vi "midiout_main.vi"() -> ()   [LabVIEW 2020]
uses:
  shared/midi note number.ctl
  midi/midi.lvclass
  0b612464-4594-4010-8acf-3e2bca421995.vi
  midi/midichannel.set.vi
  midi-ui/midi-ui.lvclass
panel:
  out "Currently Playing":T1
  out "2D Picture":picture
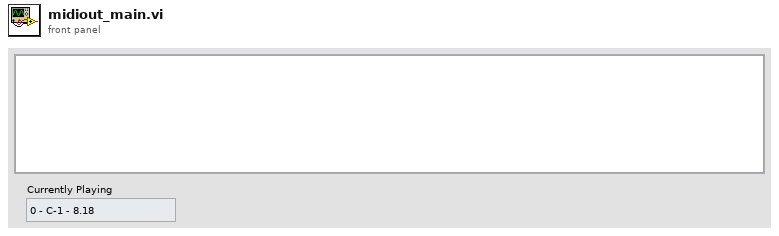
[diagram p1: front panel]
types:
  T1 = typedef "midi note number.ctl" = enum8{"0 - C-1 - 8.18", "1 - C#-1 - 8.66", "2 - D-1 - 9.18", "3 - D#-1 - 9.72", "4 - E-1 - 10.30", "5 - F-1 - 10.91", "6 - F#-1 - 11.56", "7 - G-1 - 12.25", "8 - G#-1 - 12.98", "9 - A-1 - 13.75", "10 - A#-1 - 14.57", "11 - B-1 - 15.43", "12 - C0 - 16.35", "13 - C#0 - 17.32", "14 - D0 - 18.35", "15 - D#0 - 19.45", "16 - E0 - 20.60", "17 - F0 - 21.83", "18 - F#0 - 23.12", "19 - G0 - 24.50", "20 - G#0 - 25.96", "21 - A0 - 27.50", "22 - A#0 - 29.14", "23 - B0 - 30.87", "24 - C1 - 32.70", "25 - C#1 - 34.65", "26 - D1 - 36.71", "27 - D#1 - 38.89", "28 - E1 - 41.20", "29 - F1 - 43.65", "30 - F#1 - 46.25", "31 - G1 - 49.00", "32 - G#1 - 51.91", "33 - A1 - 55.00", "34 - A#1 - 58.27", "35 - B1 - 61.74", "36 - C2 - 65.41", "37 - C#2 - 69.30", "38 - D2 - 73.42", "39 - D#2 - 77.78", "40 - E2 - 82.41", "41 - F2 - 87.31", "42 - F#2 - 92.50", "43 - G2 - 98.00", "44 - G#2 - 103.83", "45 - A2 - 110.00", "46 - A#2 - 116.54", "47 - B2 - 123.47", "48 - C3 - 130.81", "49 - C#3 - 138.59", "50 - D3 - 146.83", "51 - D#3 - 155.56", "52 - E3 - 164.81", "53 - F3 - 174.61", "54 - F#3 - 185.00", "55 - G3 - 196.00", "56 - G#3 - 207.65", "57 - A3 - 220.00", "58 - A#3 - 233.08", "59 - B3 - 246.94", "60 - C4 - 261.63", "61 - C#4 - 277.18", "62 - D4 - 293.66", "63 - D#4 - 311.13", "64 - E4 - 329.63", "65 - F4 - 349.23", "66 - F#4 - 369.99", "67 - G4 - 392.00", "68 - G#4 - 415.30", "69 - A4 - 440.00", "70 - A#4 - 466.16", "71 - B4 - 493.88", "72 - C5 - 523.25", "73 - C#5 - 554.37", "74 - D5 - 587.33", "75 - D#5 - 622.25", "76 - E5 - 659.25", "77 - F5 - 698.46", "78 - F#5 - 739.99", "79 - G5 - 783.99", "80 - G#5 - 830.61", "81 - A5 - 880.00", "82 - A#5 - 932.33", "83 - B5 - 987.77", "84 - C6 - 1046.50", "85 - C#6 - 1108.73", "86 - D6 - 1174.66", "87 - D#6 - 1244.51", "88 - E6 - 1318.51", "89 - F6 - 1396.91", "90 - F#6 - 1479.98", "91 - G6 - 1567.98", "92 - G#6 - 1661.22", "93 - A6 - 1760.00", "94 - A#6 - 1864.66", "95 - B6 - 1975.53", "96 - C7 - 2093.00", "97 - C#7 - 2217.46", "98 - D7 - 2349.32", "99 - D#7 - 2489.02", "100 - E7 - 2637.02", "101 - F7 - 2793.83", "102 - F#7 - 2959.96", "103 - G7 - 3135.96", "104 - G#7 - 3322.44", "105 - A7 - 3520.00", "106 - A#7 - 3729.31", "107 - B7 - 3951.07", "108 - C8 - 4186.01", "109 - C#8 - 4434.92", "110 - D8 - 4698.63", "111 - D#8 - 4978.03", "112 - E8 - 5274.04", "113 - F8 - 5587.65", "114 - F#8 - 5919.91", "115 - G8 - 6271.93", "116 - G#8 - 6644.88", "117 - A8 - 7040.00", "118 - A#8 - 7458.62", "119 - B8 - 7902.13", "120 - C9 - 8372.02", "121 - C#9 - 8869.84", "122 - D9 - 9397.27", "123 - D#9 - 9956.06", "124 - E9 - 10548.08", "125 - F9 - 11175.30", "126 - F#9 - 11839.82", "127 - G9 - 12543.85"}
  T2 = typedef "LVPoint32TypeDef.ctl" = cluster{"Horizontal":i32, "Vertical":i32}
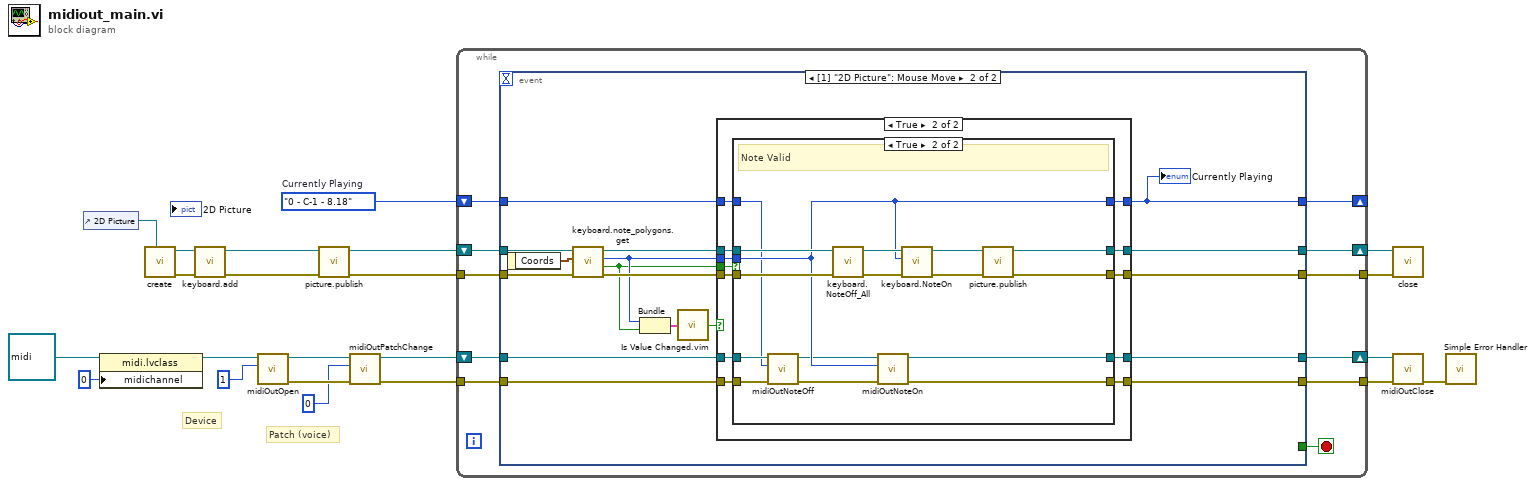
[diagram p0: block diagram]
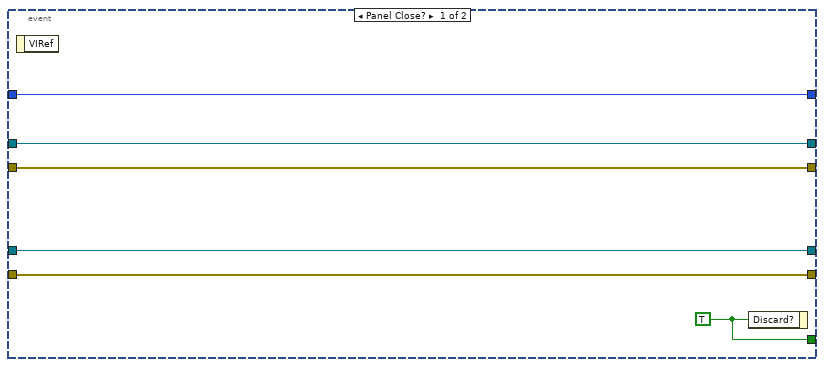
[diagram p2: hidden frame]
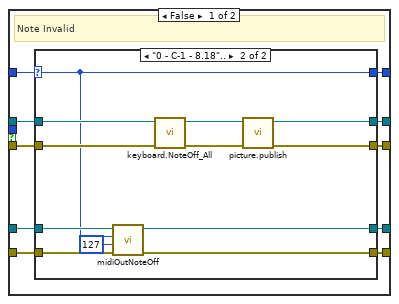
[diagram p4: hidden frame]
diagram:
  w1 = midi_note_number."0 - C-1 - 8.18"  # Currently Playing
  # "Patch (voice)"
  # "Device"
  n1 = control-ref of="2D Picture"() -> (w10:refnum<vi>)
  n2 = property class="midi.lvclass"(reference=refnum<class "midi.lvclass"> refnum ("midi in"), "midichannel"=u64 0) -> (reference out=w13:refnum<class "midi.lvclass">)  [unwired: 1 in, 1 out]
  n3 = call "create.vi"("Picture Control"=w10) -> ("error out"=w8:errorcluster, "midi-ui out"=w9:refnum<class "midi-ui.lvclass">)  [unwired: 9 in]
  n4 = call "keyboard.add.vi"("error in (no error)"=w8, "midi-ui in"=w9) -> ("error out"=w5:errorcluster, "midi-ui out"=w4:refnum<class "midi-ui.lvclass">)  [unwired: 8 in]
  n5 = call "midiOutOpen.vi"("DeviceID"=u32 1, "midi in"=w13) -> ("error out"=w18:errorcluster, "midi out"=w19:refnum<class "midi.lvclass">)  [unwired: 8 in]
  n6 = call "picture.publish.vi"("error in"=w5, "midi-ui in"=w4) -> ("error out"=w3:errorcluster, "midi-ui out"=w2:refnum<class "midi-ui.lvclass">)  [unwired: 8 in]
  n7 = call "midiOutPatchChange.vi"("error in"=w18, "Patch"=u32 0, "midi in"=w19) -> ("error out"=w6:errorcluster, "midi out"=w14:refnum<class "midi.lvclass">)  [unwired: 7 in]
  n8 = while {
    shift-right: [w29] -> w20
    shift-left: w14 -> [w28]
    tunnel: [w30] -> w12
    shift-right: [w33] -> w11
    shift-left: w2 -> [w32]
    tunnel: w3 -> [w31]
    tunnel: [w27] -> w7
    tunnel: w6 -> [w26]
    shift-right: [w24] -> _
    shift-left: w1 -> [w23]
    stop <- w25 stop-if-true
    n9 = event shown="[1] \"2D Picture\": Mouse Move" {
      selector: _ -> [_ _]
      dyn-events: _ -> [_ _]
      timeout: _ -> [_ _]
      tunnel: [w39 w47] -> w33
      tunnel: w32 -> [w39 w55]
      tunnel: w31 -> [w38 w54]
      tunnel: [w38 w46] -> w30
      tunnel: [w37 w49] -> w29
      tunnel: w28 -> [w37 w51]
      tunnel: [w36 w48] -> w27
      tunnel: w26 -> [w36 w50]
      tunnel: [w35 _] -> w25
      tunnel: [w34 w40] -> w24
      tunnel: w23 -> [w34 w41]
      event Panel Close? {
        w35 = TRUE ("Discard?")
        n10 = event-data() -> ()  [unwired: 1 in, 1 out]
        n11 = event-data("Discard?"=w35) -> ()  [unwired: 1 in, 1 out]
      }
      event "2D Picture": Mouse Move {
        n12 = event-data() -> ("Coords"=w56:T2)  [unwired: 1 in]
        n13 = call "keyboard.note_polygons.get.vi"("error in (no error)"=w54, "Cursor Position"=w56, "midi-ui in"=w55) -> ("error out"=w52:errorcluster, "Valid"=w42:bool, "Note"=w45:T1, "midi-ui out"=w53:refnum<class "midi-ui.lvclass">)  [unwired: 5 in]
        n14 = Bundle("Note"=w45, "Valid"=w42) -> (w44:cluster{"Note":T1, "Valid":bool})  [unwired: 1 in]
        n15 = call "Is Value Changed.vim"("value"=w44) -> ("changed or first call?"=w43:bool)
        n16 = case shown="True" w43 {
          tunnel: w53 -> [w61 w73]
          tunnel: w52 -> [w60 w72]
          tunnel: w51 -> [w59 w71]
          tunnel: w50 -> [w58 w70]
          tunnel: [w57 w69] -> w40
          tunnel: [w59 w68] -> w49
          tunnel: [w58 w67] -> w48
          tunnel: [w61 w66] -> w47
          tunnel: [w60 w65] -> w46
          tunnel: w45 -> [_ w64]
          tunnel: w42 -> [_ w63]
          tunnel: w41 -> [w57 w62]
          frame False {
          }
          frame True {
            n17 = case shown="True" w63 {
              tunnel: w73 -> [w83 w110]
              tunnel: w72 -> [w82 w107]
              tunnel: w71 -> [w81 w105]
              tunnel: w70 -> [w80 w104]
              tunnel: [w75 w106] -> w69
              tunnel: [w79 w114] -> w68
              tunnel: [w78 w113] -> w67
              tunnel: [w77 w116] -> w66
              tunnel: [w76 w115] -> w65
              tunnel: w64 -> [_ w106]
              tunnel: w62 -> [w74 w101]
              frame False {
                # "Note Invalid"
                n18 = case shown="\"0 - C-1 - 8.18\".." w74 {
                  selector: w74 -> [w88 w90]
                  tunnel: w83 -> [w87 w94]
                  tunnel: w82 -> [w86 w93]
                  tunnel: w81 -> [w85 w100]
                  tunnel: w80 -> [w84 w99]
                  tunnel: [w88 w90] -> w75
                  tunnel: [w85 w98] -> w79
                  tunnel: [w84 w97] -> w78
                  tunnel: [w87 w96] -> w77
                  tunnel: [w86 w95] -> w76
                  frame Default {
                  }
                  frame "0 - C-1 - 8.18".. {
                    n19 = call "midiOutNoteOff.vi"("error in"=w99, "Velocity (0-127)"=127, "Note"=w90, "midi in"=w100) -> ("error out"=w97:errorcluster, "midi out"=w98:refnum<class "midi.lvclass">)  [unwired: 6 in]
                    n20 = call "keyboard.NoteOff_All.vi"("error in (no error)"=w93, "midi-ui in"=w94) -> ("error out"=w91:errorcluster, "midi-ui out"=w92:refnum<class "midi-ui.lvclass">)  [unwired: 8 in]
                    n21 = call "picture.publish.vi"("error in"=w91, "midi-ui in"=w92) -> ("error out"=w95:errorcluster, "midi-ui out"=w96:refnum<class "midi-ui.lvclass">)  [unwired: 8 in]
                  }
                }
              }
              frame True {
                # "Note Valid"
                n22 = call "midiOutNoteOff.vi"("error in"=w104, "Note"=w101, "midi in"=w105) -> ("error out"=w103:errorcluster, "midi out"=w102:refnum<class "midi.lvclass">)  [unwired: 7 in]
                n23 = call "keyboard.NoteOff_All.vi"("error in (no error)"=w107, "midi-ui in"=w110) -> ("error out"=w108:errorcluster, "midi-ui out"=w109:refnum<class "midi-ui.lvclass">)  [unwired: 8 in]
                n24 = call "midiOutNoteOn.vi"("error in"=w103, "Note"=w106, "midi in"=w102) -> ("error out"=w113:errorcluster, "midi out"=w114:refnum<class "midi.lvclass">)  [unwired: 7 in]
                n25 = call "keyboard.NoteOn.vi"("error in (no error)"=w108, "Note"=w106, "midi-ui in"=w109) -> ("error out"=w111:errorcluster, "midi-ui out"=w112:refnum<class "midi-ui.lvclass">)  [unwired: 7 in]
                n26 = call "picture.publish.vi"("error in"=w111, "midi-ui in"=w112) -> ("error out"=w115:errorcluster, "midi-ui out"=w116:refnum<class "midi-ui.lvclass">)  [unwired: 8 in]
              }
            }
          }
        }
        "Currently Playing" <- w40
      }
    }
  }
  n27 = call "close.vi"("error in (no error)"=w12, "midi-ui in"=w11) -> ()  [unwired: 9 in, 1 out]
  n28 = call "midiOutClose.vi"("error in"=w7, "midi in"=w20) -> ("error out"=w22:errorcluster)  [unwired: 8 in, 1 out]
  n29 = call <vilib>:"Simple Error Handler.vi"("error in (no error)"=w22) -> ()  [unwired: 4 in, 5 out]
